vi "RFH-convert-avg-libreVNA.vi"(5 "average filepath":path, 7 "Source Folder":path, 8 "error in (no error)":errorcluster, 10 "Frequency low":dbl=1000000000.0) -> (0 "error out":errorcluster, 2 "Common Format":T1)   [LabVIEW 2020, in "RFH-Reflection_File_Handler.lvlib"]
doc: "Averages the LibreVNA files of a folder, removes data below the low frequency and saves the result as a common-format file."
uses:
  RFH-Reflection_File_Handler.lvlib
  RFH-common_data_format.ctl
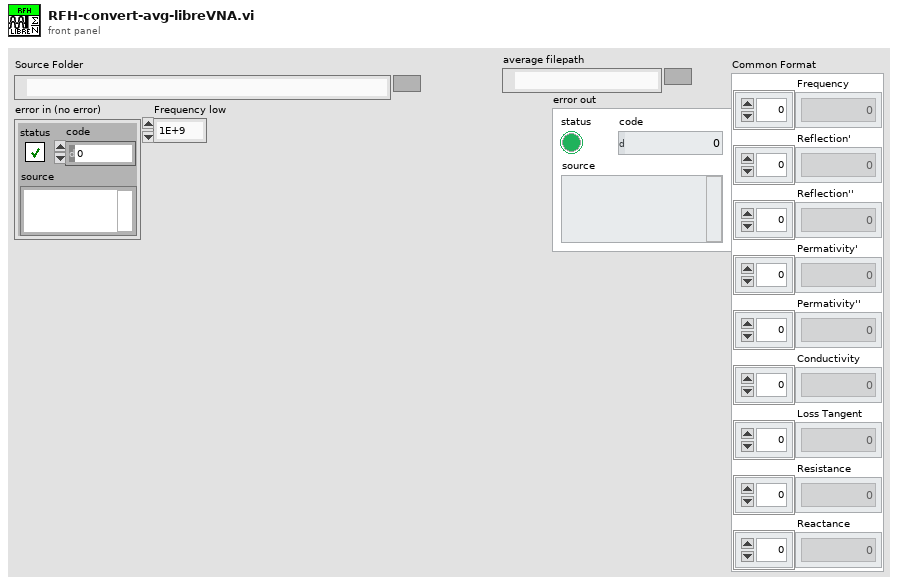
[diagram p1: front panel]
types:
  T1 = typedef "RFH-Reflection_File_Handler.lvlib/RFH-common_data_format.ctl" = cluster{"Frequency":dbl[], "Reflection'":dbl[], "Reflection''":dbl[], "Permativity'":dbl[], "Permativity''":dbl[], "Conductivity":dbl[], "Loss Tangent":dbl[], "Resistance":dbl[], "Reactance":dbl[]}
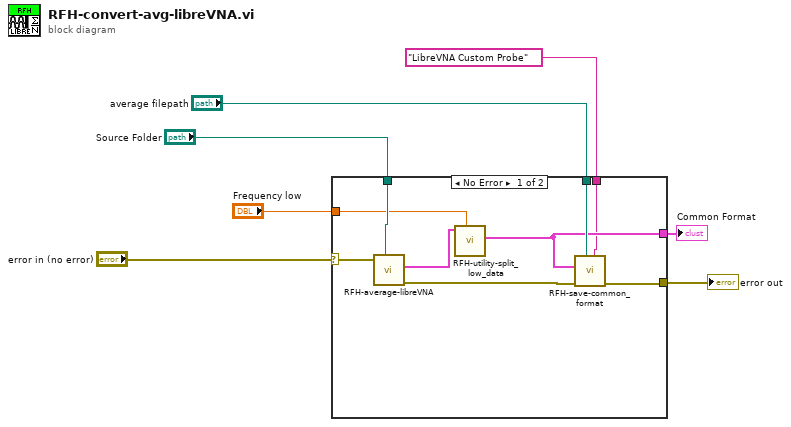
[diagram p0: block diagram]
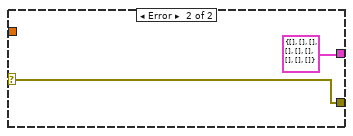
[diagram p2: hidden frame]
diagram:
  n1 = case shown="No Error" "error in (no error)" {
    selector: "error in (no error)" -> [w14 w18]
    tunnel: "Source Folder" -> [w13 _]
    tunnel: "average filepath" -> [w16 _]
    tunnel: [w15 w18] -> w4
    tunnel: [w9 T1 {"Frequency"=[], "Reflection'"=[], "Reflection''"=[], "Permativity'"=[], "Permativity''"=[], "Conductivity"=[], "Loss Tangent"=[], "Resistance"=[], "Reactance"=[]} ("Common Format")] -> w3
    tunnel: "Frequency low" -> [w11 _]
    tunnel: "LibreVNA Custom Probe" ("source") -> [w8 _]
    frame No Error {
      n2 = call "RFH-average-libreVNA.vi"("Source Folder"=w13, "error in (no error)"=w14) -> ("error out"=w12:errorcluster, "Common Format"=w10:T1)  [unwired: 8 in]
      n3 = call "RFH-utility-split_low_data.vi"("Frequency"=w11, "Common Format"=w10) -> ("After"=w9:T1)  [unwired: 9 in]
      n4 = call "RFH-save-common_format.vi"("source"=w8, "file path (use dialog)"=w16, "error in (no error)"=w12, "Common Format"=w9) -> ("error out"=w15:errorcluster)  [unwired: 7 in]
    }
    frame Error {
    }
  }
  "error out" <- w4
  "Common Format" <- w3
